vi "while_st.vi"() -> ()   [LabVIEW 2020]
uses:
  <vilib>/Utility/error.llb/Error Cluster From Error Code.vi
panel:
  in  "ClusterZ":cluster{"NumZ":dbl}
  in  "ClusterY":cluster{"NumY":dbl}
  out "W4Count":bool
  out "W3Count":bool
  out "W2Count":bool
  out "CountOut":dbl
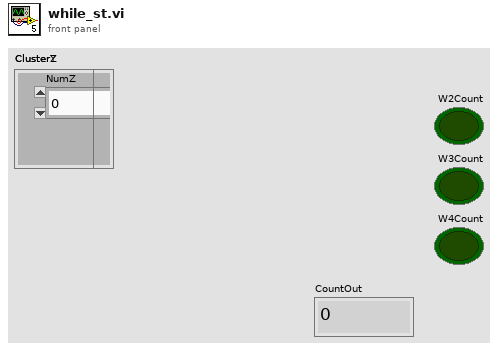
[diagram p1: front panel]
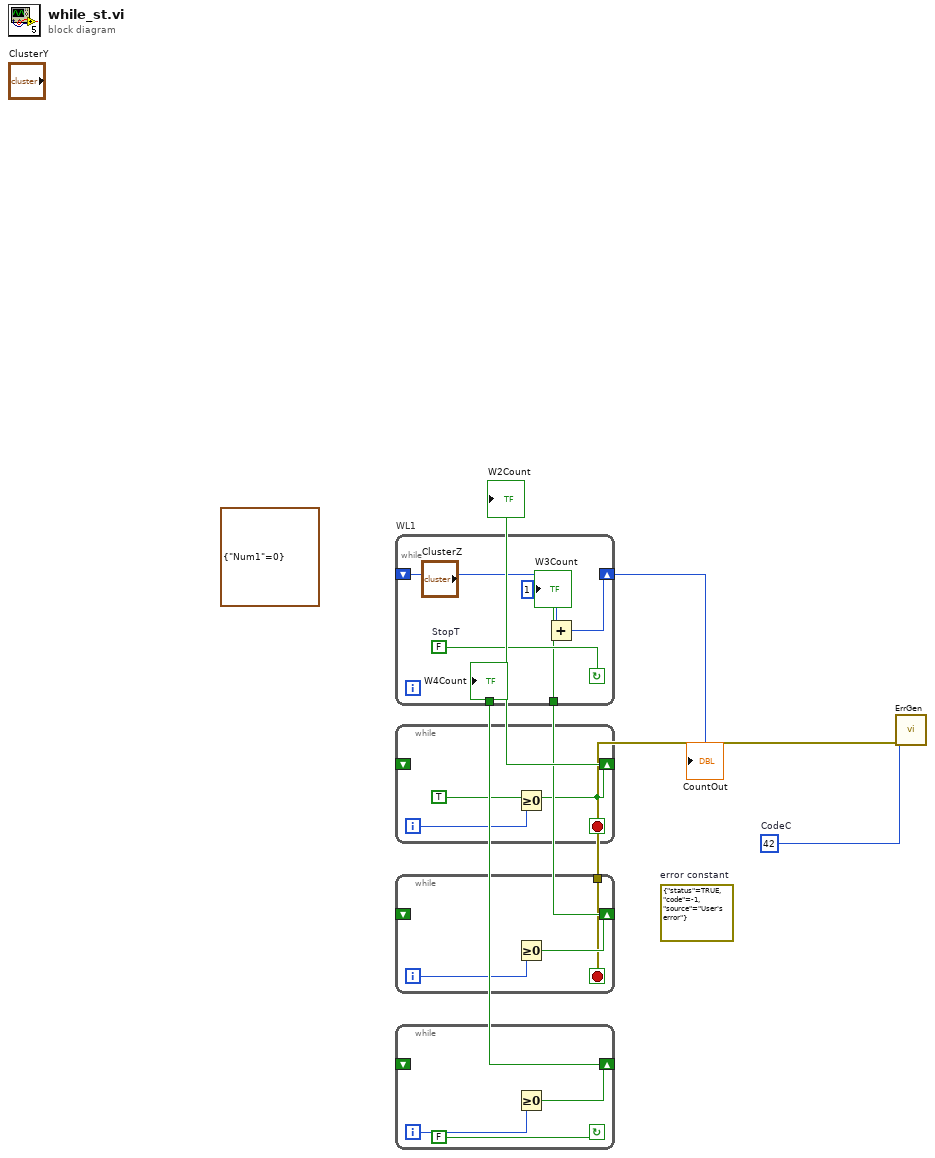
[diagram p0: block diagram]
diagram:
  (unwired) cluster{"Num1":i32} {"Num1"=0} ("clusterX")
  w3 = 42  # CodeC
  (unwired) errorcluster {"status"=TRUE, "code"=-1, "source"="User's error"}  # error constant
  n1 = while "WL2" {
    shift-right: [w7] -> w5
    shift-left: _ -> [_]
    i -> [w8]
    stop <- w7 stop-if-true
    w7 = TRUE ("BoolT")
    n2 = Greater Or Equal To 0? ("GE2")(x=w8) -> ()  [unwired: 1 out]
  }
  "W2Count" <- w5
  n3 = while "WL4" {
    shift-right: [w10] -> w1
    shift-left: _ -> [_]
    i -> [w9]
    stop <- FALSE ("StopF") continue-if-true
    n4 = Greater Or Equal To 0? ("GE4")(x=w9) -> (x >= 0?=w10:bool)
  }
  n5 = call "ErrGen"("error code (0)"=w3) -> ("error out"=w2:errorcluster)  [unwired: 8 in]
  n6 = while "WL3" {
    shift-right: [w13] -> w4
    shift-left: _ -> [_]
    tunnel: w2 -> [w12]
    i -> [w14]
    stop <- w12 stop-if-true
    n7 = Greater Or Equal To 0? ("GE3")(x=w14) -> (x >= 0?=w13:bool)
  }
  n8 = while "WL1" {
    shift-right: [w17] -> w6
    shift-left: _ -> [w19]
    tunnel: w4 -> [w16]
    tunnel: w1 -> [w15]
    stop <- w20 continue-if-true
    w20 = FALSE  # StopT
    n9 = Add ("Add1")(x=w19, y=1 ("OneC")) -> (x+y=w17:i32)
    "W3Count" <- w16
    "W4Count" <- w15
  }
  "CountOut" <- w6
